vi "Parse NSA Call Handover Param.vi"(8 "error in (no error)":errorcluster caption="에러 입력(에러 없음)", 10 "JSON string":string, 11 "Instrument Manager 입력":refnum<class "Instrument Manager.lvclass">) -> (0 "error out":errorcluster caption="에러 출력", 1 "NSA Call Handover Param":T2, 2 "Call Handover Param LTE":T1, 3 "Instrument Manager 출력":refnum<class "Instrument Manager.lvclass">)   [LabVIEW 2023, in "Instrument Manager.lvclass"]
uses:
  Instrument Manager.lvclass
  Type Definition/NSA Call Handover Param.ctl
  Module/ANRITSU Call Box/Type Definition/NR Modulation Type.ctl
  Param Definition/Call Handover Param NSA.ctl
  Instrument Manager.lvclass/Instrument Manager.ctl
  Module/ANRITSU Call Box/ANRITSU Call Box.lvlib
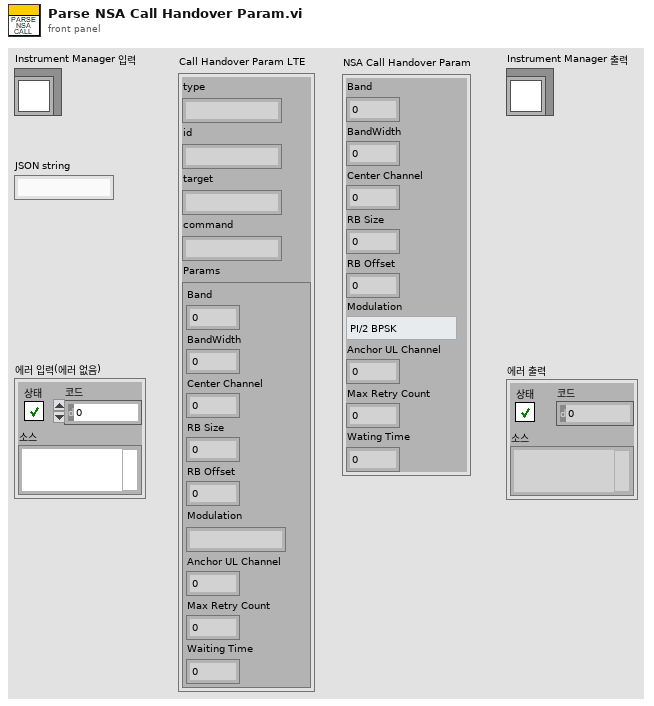
[diagram p1: front panel]
types:
  T1 = typedef "Instrument Manager.lvclass/Call Handover Param NSA.ctl" = cluster{"type":string, "id":string, "target":string, "command":string, "Params":cluster{"Band":u32, "BandWidth":u32, "Center Channel":u32, "RB Size":i32, "RB Offset":i32, "Modulation":string, "Anchor UL Channel":i32, "Max Retry Count":i32, "Waiting Time":i32}}
  T2 = typedef "NSA Call Handover Param.ctl" = cluster{"Band":u32, "BandWidth":u32, "Center Channel":u32, "RB Size":i32, "RB Offset":i32, "Modulation":T3, "Anchor UL Channel":i32, "Max Retry Count":i32, "Wating Time":i32}
  T3 = typedef "ANRITSU Call Box.lvlib/NR Modulation Type.ctl" = enum16{"PI/2 BPSK", "QPSK", "16QAM", "64QAM", "256QAM"}
  T4 = cluster{"Band":u32, "BandWidth":u32, "Center Channel":u32, "RB Size":i32, "RB Offset":i32, "Modulation":string, "Anchor UL Channel":i32, "Max Retry Count":i32, "Waiting Time":i32}
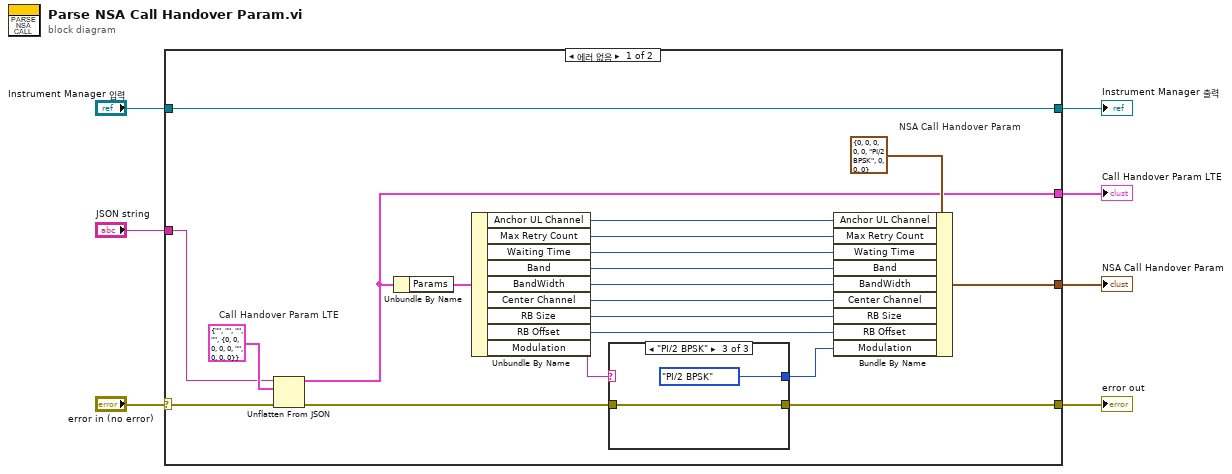
[diagram p0: block diagram]
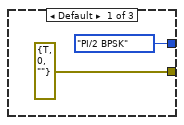
[diagram p2: hidden frame]
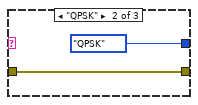
[diagram p3: hidden frame]
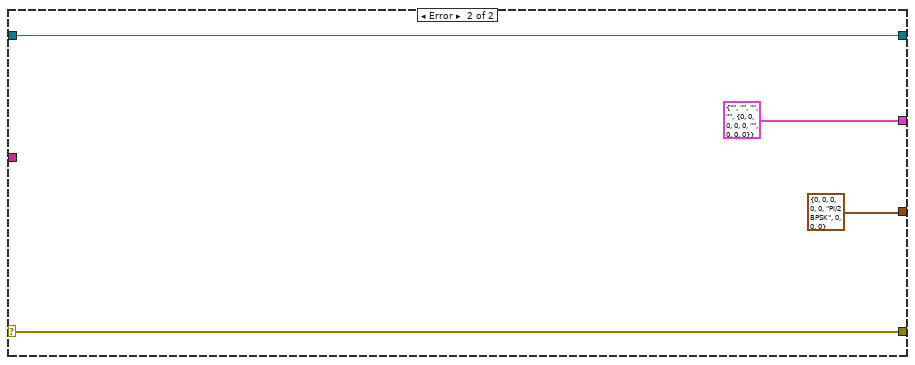
[diagram p4: hidden frame]
diagram:
  n1 = case shown="에러 없음" "error in (no error)" {
    selector: "error in (no error)" -> [w15 w37]
    tunnel: [w12 w37] -> w6
    tunnel: [w27 w36] -> w4
    tunnel: "Instrument Manager 입력" -> [w27 w36]
    tunnel: [w11 T2 {"Band"=0, "BandWidth"=0, "Center Channel"=0, "RB Size"=0, "RB Offset"=0, "Modulation"=enum."PI/2 BPSK", "Anchor UL Channel"=0, "Max Retry Count"=0, "Wating Time"=0} ("NSA Call Handover Param")] -> w3
    tunnel: [w10 T1 {"type"="", "id"="", "target"="", "command"="", "Params"={"Band"=0, "BandWidth"=0, "Center Channel"=0, "RB Size"=0, "RB Offset"=0, "Modulation"="", "Anchor UL Channel"=0, "Max Retry Count"=0, "Waiting Time"=0}} ("Call Handover Param LTE")] -> w2
    tunnel: "JSON string" -> [w9 _]
    frame No Error {
      w13 = T2 {"Band"=0, "BandWidth"=0, "Center Channel"=0, "RB Size"=0, "RB Offset"=0, "Modulation"=enum."PI/2 BPSK", "Anchor UL Channel"=0, "Max Retry Count"=0, "Wating Time"=0}  # NSA Call Handover Param
      w14 = T1 {"type"="", "id"="", "target"="", "command"="", "Params"={"Band"=0, "BandWidth"=0, "Center Channel"=0, "RB Size"=0, "RB Offset"=0, "Modulation"="", "Anchor UL Channel"=0, "Max Retry Count"=0, "Waiting Time"=0}}  # Call Handover Param LTE
      n2 = Unflatten From JSON(JSON string=w9, type and defaults=w14, error in (no error)=w15) -> (value=w10:T1, error out=w18:errorcluster)  [unwired: 4 in]
      n3 = Unbundle By Name(w10) -> ("Params"=w26:T4)
      n4 = Unbundle By Name(w26) -> ("Anchor UL Channel"=w8:i32, "Max Retry Count"=w16:i32, "Waiting Time"=w24:i32, "Band"=w23:u32, "BandWidth"=w22:u32, "Center Channel"=w21:u32, "RB Size"=w20:i32, "RB Offset"=w19:i32, "Modulation"=w25:string)
      n5 = case shown="\"PI/2 BPSK\"" w25 {
        tunnel: w18 -> [_ w30 w32]
        tunnel: [NR_Modulation_Type."PI/2 BPSK" ("Modulation") NR_Modulation_Type."QPSK" ("Modulation") NR_Modulation_Type."PI/2 BPSK" ("Modulation")] -> w17
        tunnel: [errorcluster {"status"=TRUE, "code"=0, "source"=""} ("error out") w30 w32] -> w12
        frame Default {
        }
        frame "QPSK" {
        }
        frame "PI/2 BPSK" {
        }
      }
      n6 = Bundle By Name(cluster=w13, "Anchor UL Channel"=w8, "Max Retry Count"=w16, "Wating Time"=w24, "Band"=w23, "BandWidth"=w22, "Center Channel"=w21, "RB Size"=w20, "RB Offset"=w19, "Modulation"=w17) -> (w11:T2)
    }
    frame Error {
    }
  }
  "error out" <- w6
  "Instrument Manager 출력" <- w4
  "NSA Call Handover Param" <- w3
  "Call Handover Param LTE" <- w2
